vi "SMR_LabVIEW_V9.vi"() -> ()   [LabVIEW 2025]
uses:
  <vilib>/DAQmx/write.llb/DAQmx Write (Analog DBL 1Chan 1Samp).vi
  <vilib>/DAQmx/read.llb/DAQmx Read (Analog 1D DBL NChan 1Samp).vi
  <vilib>/DAQmx/read.llb/DAQmx Read (Analog 2D DBL NChan NSamp).vi
  <vilib>/Analysis/baseanly.llb/Mean (DBL).vi
  <vilib>/DAQmx/create/channels.llb/DAQmx Create Channel (AI-Temperature-Thermocouple).vi
  <vilib>/DAQmx/create/channels.llb/DAQmx Create Channel (AI-Voltage-Basic).vi
  <vilib>/DAQmx/create/channels.llb/DAQmx Create Channel (AO-Voltage-Basic).vi
  <vilib>/DAQmx/miscellaneous.llb/DAQmx Fill In Error Info.vi
  <vilib>/DAQmx/configure/timing.llb/DAQmx Timing (Sample Clock).vi
  <vilib>/addons/control/pid/pid.llb/PID (DBL).vi
  <vilib>/measure/maspectr.llb/FFT Power Spectrum and PSD for 1 Chan.vi
  <vilib>/measure/matone.llb/Extract Single Tone Information 1 Chan.vi
  <vilib>/addons/control/pid/NI_PID_pid.lvlib
  <vilib>/Analysis/NI_AALBase.lvlib
  <vilib>/ptbypt/NI_PtbyPt.lvlib
  <vilib>/measure/NI_MAPro.lvlib
panel:
  out "Room Temp (deg C)":dbl
  out "HW Valve Command (V)":dbl
  in  "HX Flow Setpoint (GPM)":dbl
  in  "Manual HW Valve Voltage (V)":dbl
  in  "HW Valve: Manual / PID":bool
  in  "PID gains for HW Valve":T1={"proportional gain (Kc)"=1.0, "integral time (Ti, min)"=0.01, "derivative time (Td, min)"=0.0} {"derivative time (Td, min)" format="%.3f"; "integral time (Ti, min)" format="%.3f"; "proportional gain (Kc)" format="%.3f"}
  out "Rod Power (W)":dbl
  out "Current Through Rod (A)":dbl
  out "Time in Steady State (s)":dbl
  in  "Steady-State Dwell (s)":dbl
  out "Main Loop Flow (GPM)":dbl
  out "FM Amplitude":dbl
  out "FM Frequency":dbl
  out "Spectrum":cluster{"f0":dbl, "df":dbl, "magnitude":dbl[]}(graph)
  out "Raw Signal":waveform(dbl)(graph)
  out "Smoothed HX Flow (GPM)":dbl
  out "Flow History":dbl(graph)
  out "HX Flow (GPM)":dbl
  out "Voltage Across Rod (V)":dbl format="%0.2f"
  out "Current Run Folder":path
  in  "Log Root Folder":path=path "C:/Users/LocalUser/Documents/GitHub/thermal-loop/resources/v0.1.1/data/001"
  out "Raw NI9201 \nVoltage Display":T2
  in  "Loop Period (ms)":dbl=1000.0
  in  "Stop":bool
  out "Auto Steady State Threshold (deg C/min)":dbl
  out "Max dT/dt (deg C/min)":dbl
  out "Temp Change Rate (deg C/min)":dbl
  out "5-Min Baseline Complete":bool
  out "Rate Window Ready":bool
  out "Steady State":bool
  in  "Voltage Limit (V)":dbl=10.0
  in  "Temperature Limit (C)":dbl=50.0
  in  "Pressure Limit (psi)":dbl=15.0
  out "Max Voltage":bool
  out "Max Temperature":bool
  out "Max Pressure":bool
  out "Heat Exchanger Pressure History":dbl(graph)
  out "Main Loop Pressure History":T3(graph)
  out "Overall Avg Pressure (psi)":dbl
  out "Heat Exchanger Pressure P6 (psi)":dbl
  out "Main Loop Avg Pressure (psi)":dbl
  out "Pressure Display":T4
  out "Overall Pressure History":T5(graph)
  out "Max Loop Pressure (psi)":dbl
  out "Heat Exchanger Temperature History":cluster{"Waveform":dbl, "Waveform":dbl}(graph)
  out "Main Loop Temeperature History":T6(graph)
  out "Heat Exchanger Avg Temp (deg C)":dbl
  out "Temperature Display":T7
  out "Overall Temperature History":T8(graph)
  out "Overall Avg Temp (deg C)":dbl
  out "Max Loop Temp (deg C)":dbl
  out "Final P-Valve Voltage (V)":dbl
  out "PID Trim Voltage (V)":dbl
  in  "PID Temp Setpoint (deg C)":dbl
  in  "Auto PID Enable":bool
  in  "Manual P-Valve Voltage (V)":dbl min=0.0 max=10.0
  out "Main Loop Avg Temp (deg C)":dbl
  # "HoneyWell Valve Control"
  # "Heat Exchanger Flow"
  # "Control/Troubleshoot"
  # "Steady State"
  # "Emergency Indicators"
  # "Pressure"
  # "Temperature"
  # "Proportional Valve Control"
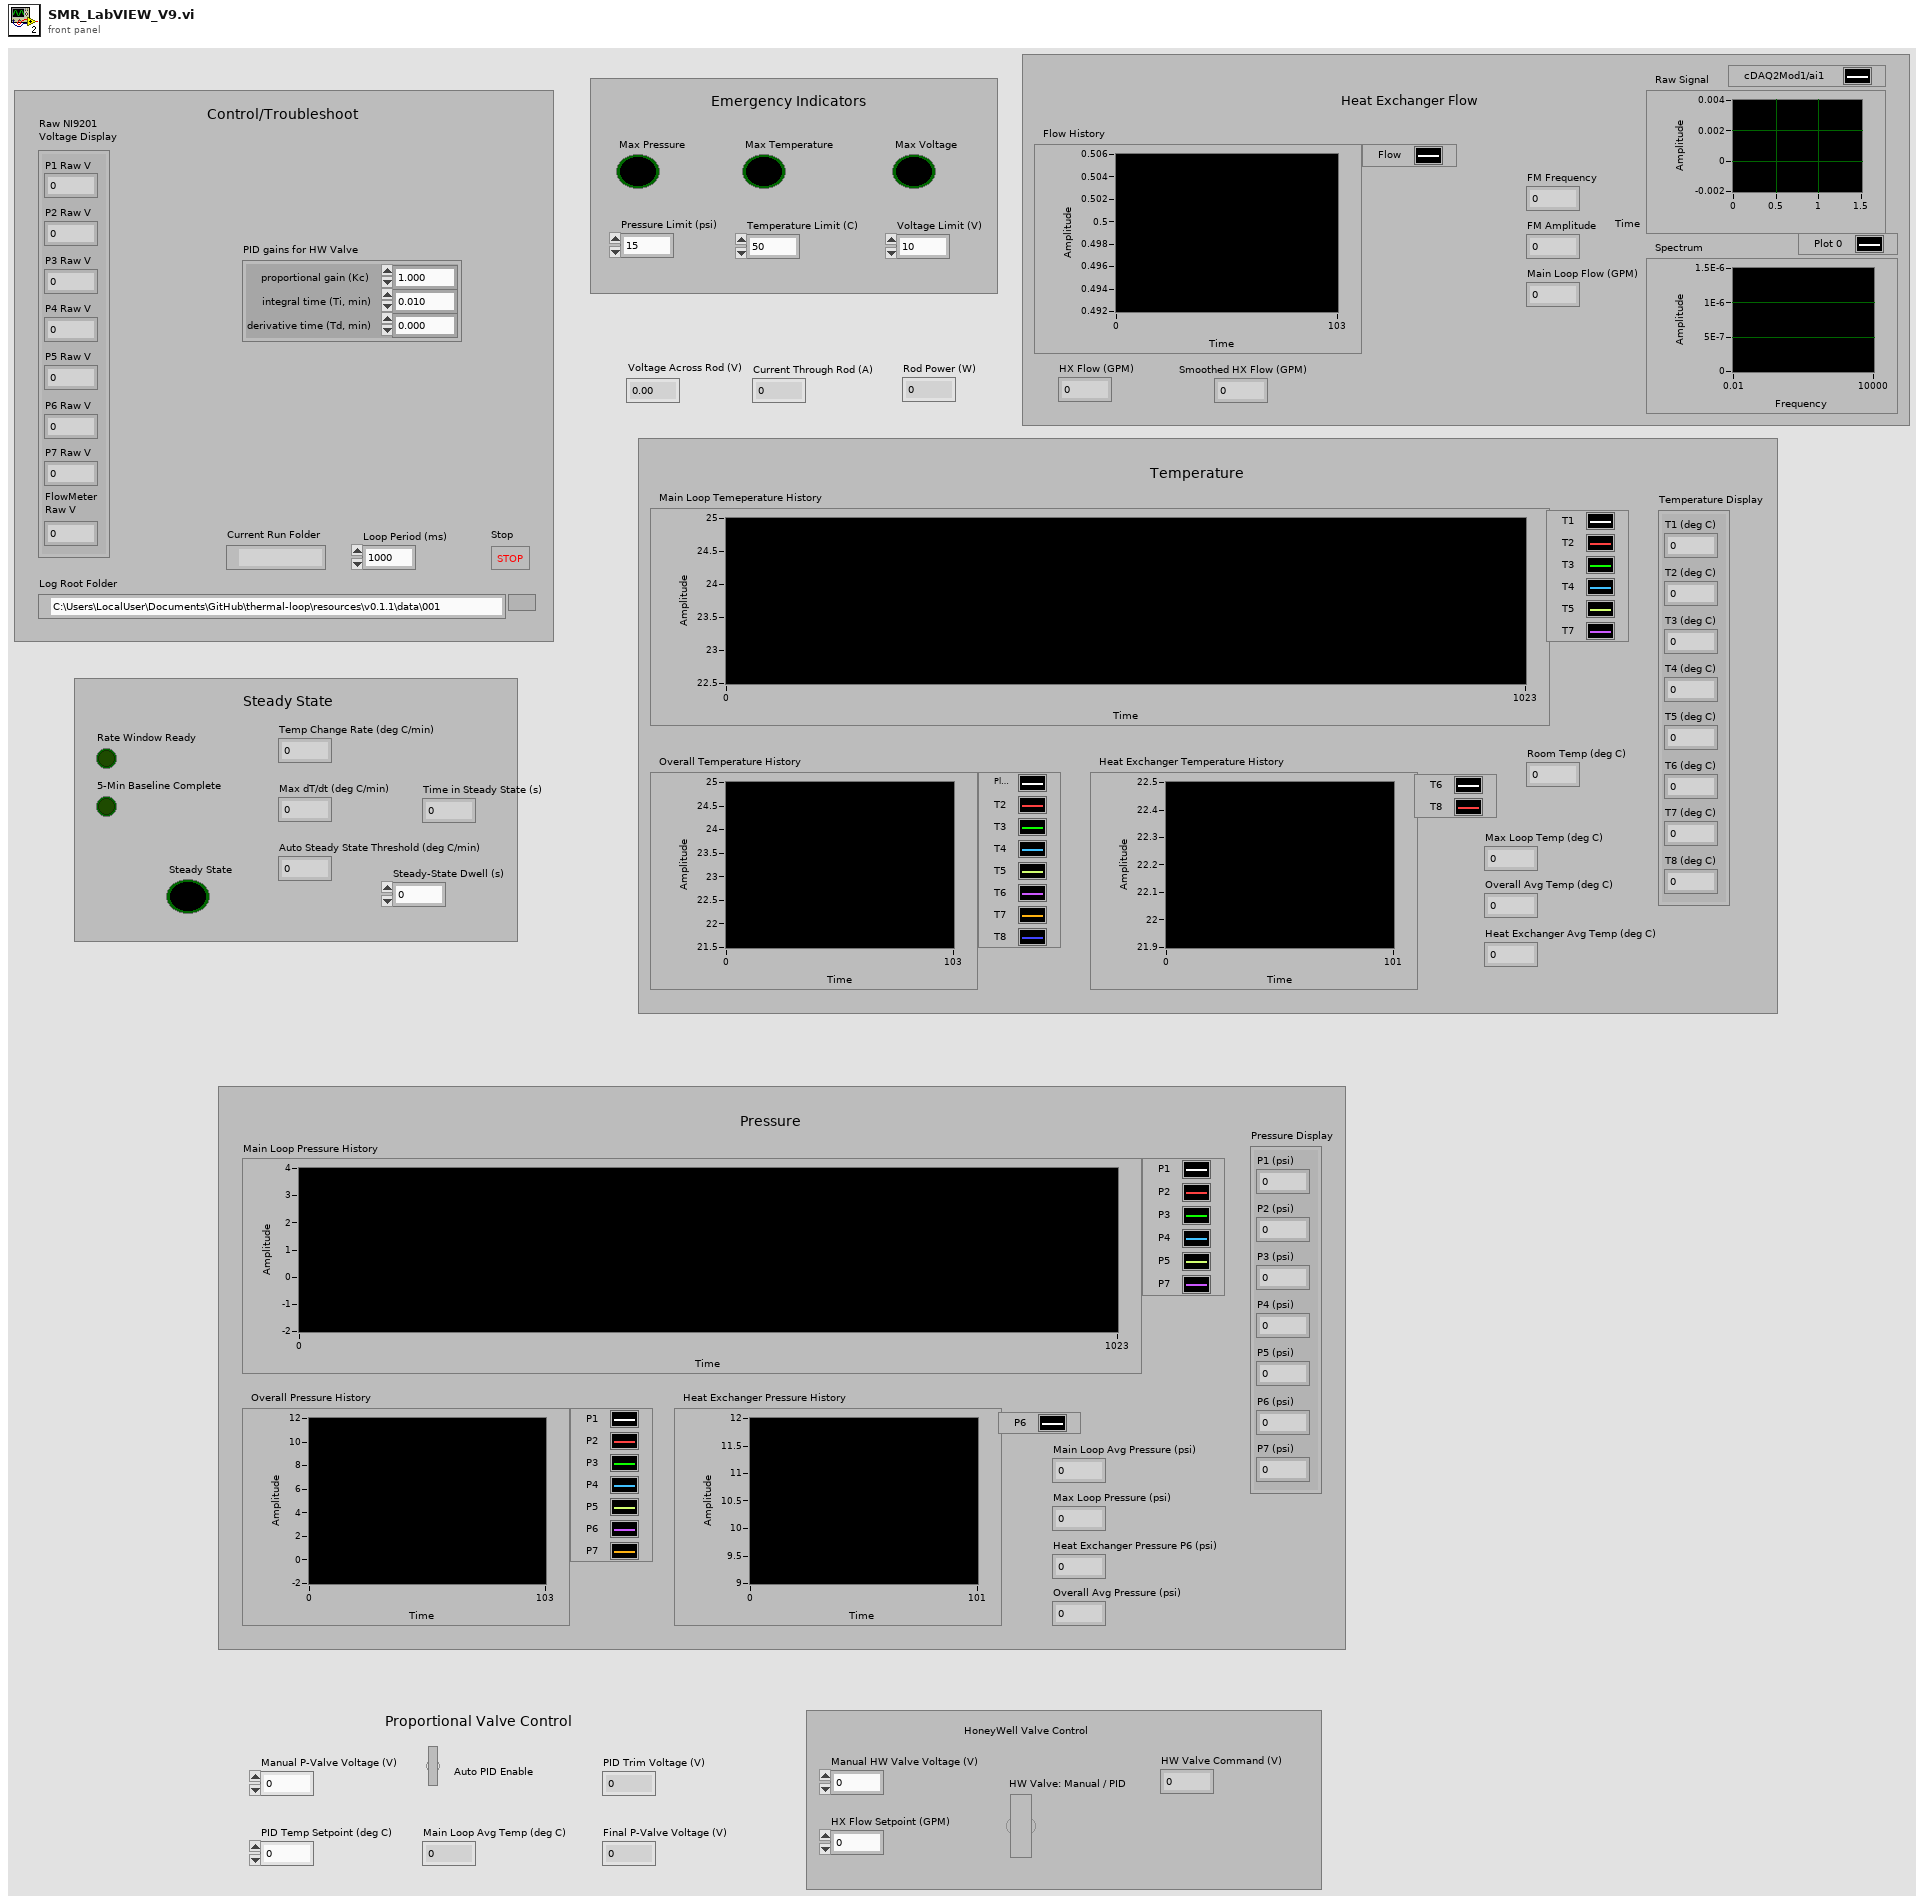
[diagram p1: front panel]
types:
  T1 = cluster{"proportional gain (Kc)":dbl, "integral time (Ti, min)":dbl, "derivative time (Td, min)":dbl}
  T2 = cluster{"P1 Raw V":dbl, "P2 Raw V":dbl, "P3 Raw V":dbl, "P4 Raw V":dbl, "P5 Raw V":dbl, "P6 Raw V":dbl, "P7 Raw V":dbl, "FlowMeter\nRaw V":dbl}
  T3 = cluster{"P1":dbl, "P2":dbl, "P3":dbl, "P4":dbl, "P5":dbl, "P7":dbl}
  T4 = cluster{"P1 (psi)":dbl, "P2 (psi)":dbl, "P3 (psi)":dbl, "P4 (psi)":dbl, "P5 (psi)":dbl, "P6 (psi)":dbl, "P7 (psi)":dbl}
  T5 = cluster{"P1":dbl, "P2":dbl, "P3":dbl, "P4":dbl, "P5":dbl, "P6":dbl, "P7":dbl}
  T6 = cluster{"Waveform":dbl, "Waveform":dbl, "Waveform":dbl, "Waveform":dbl, "Waveform":dbl, "Waveform":dbl}
  T7 = cluster{"T1 (deg C)":dbl, "T2 (deg C)":dbl, "T3 (deg C)":dbl, "T4 (deg C)":dbl, "T5 (deg C)":dbl, "T6 (deg C)":dbl, "T7 (deg C)":dbl, "T8 (deg C)":dbl}
  T8 = cluster{"Waveform":dbl, "Waveform":dbl, "Waveform":dbl, "Waveform":dbl, "Waveform":dbl, "Waveform":dbl, "Waveform":dbl, "Waveform":dbl}
  T9 = enum16{"open", "replace", "create", "open or create", "replace or create", "replace or create with confirmation"}
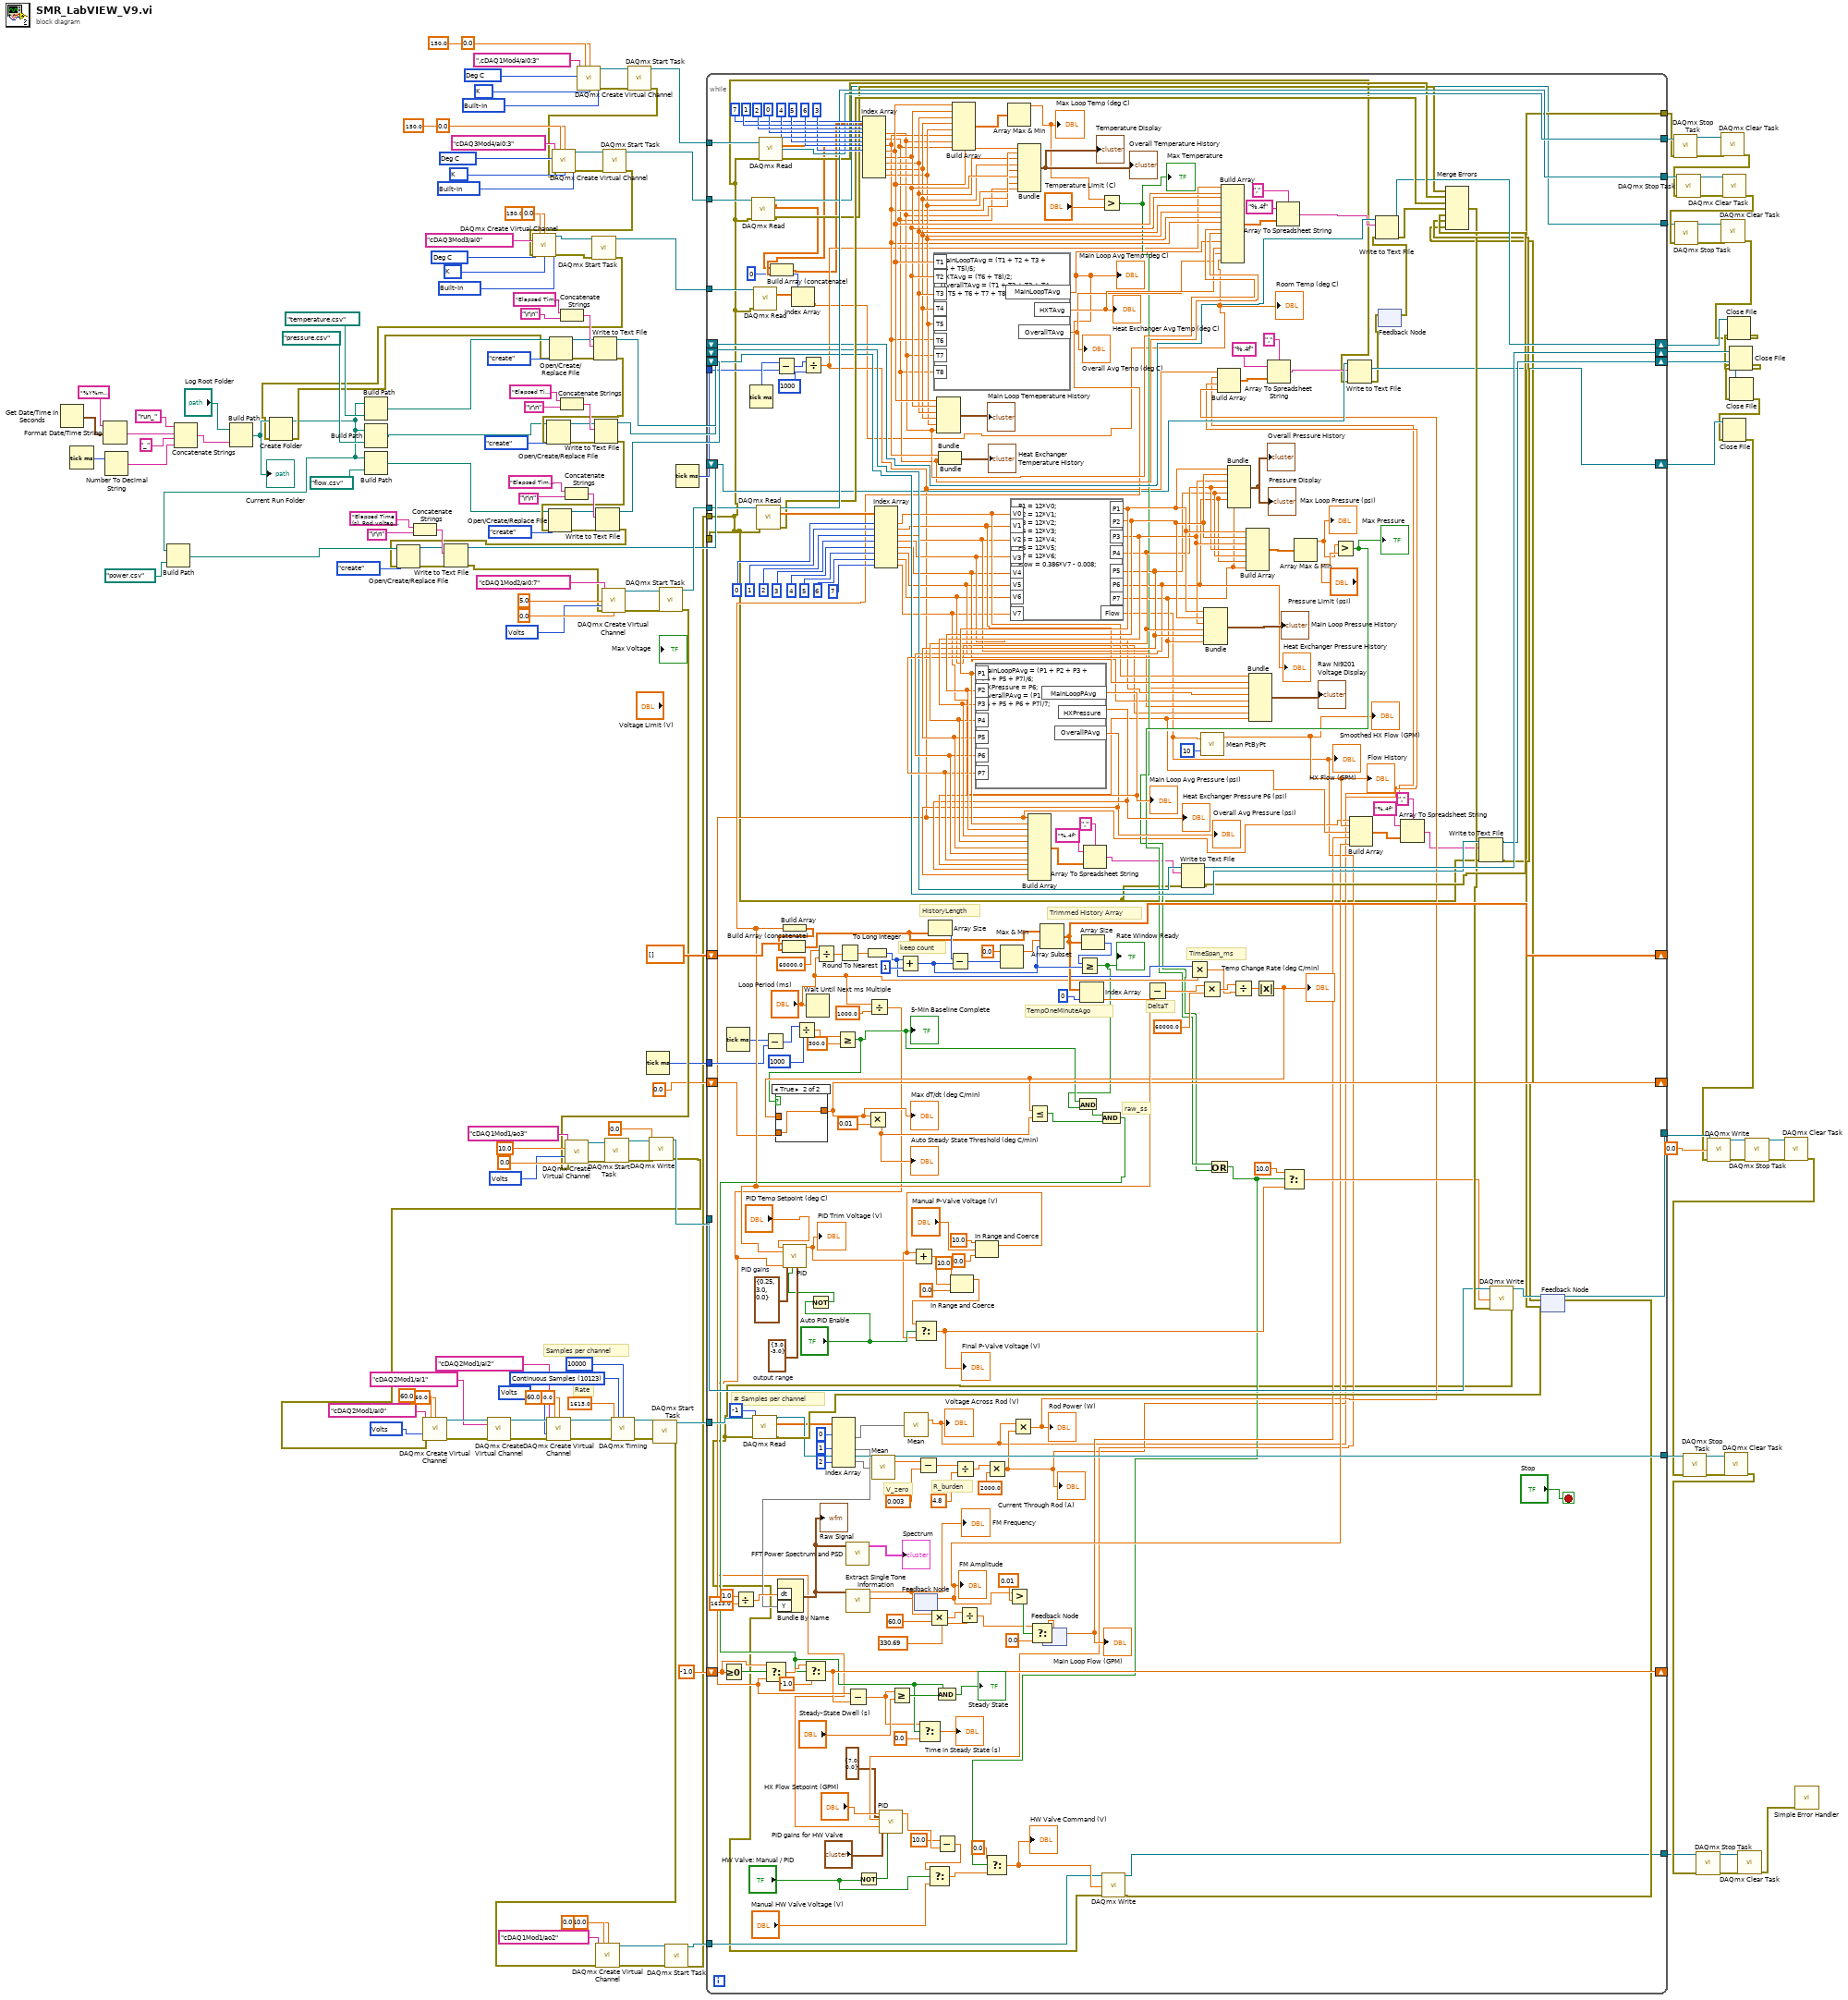
[diagram p0: block diagram]
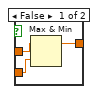
[diagram p2: hidden frame]
diagram:
  w1 = 10200 items=["Built-In"=10200, "Constant Value"=10116, "Channel"=10113] ("cjc source")
  w2 = 10073 items=["J"=10072, "K"=10073, "N"=10077, "R"=10082, "S"=10085, "T"=10086, "B"=10047, "E"=10055] ("thermocouple type")
  w8 = 10143 items=["Deg C"=10143, "Deg F"=10144, "Kelvins"=10325, "Deg R"=10145, "From Custom Scale"=10065] ("units")
  w28 = 10348 items=["Volts"=10348, "From Custom Scale"=10065] ("units")
  w44 = 10200 items=["Built-In"=10200, "Constant Value"=10116, "Channel"=10113] ("cjc source")
  w45 = 10073 items=["J"=10072, "K"=10073, "N"=10077, "R"=10082, "S"=10085, "T"=10086, "B"=10047, "E"=10055] ("thermocouple type")
  w46 = 10143 items=["Deg C"=10143, "Deg F"=10144, "Kelvins"=10325, "Deg R"=10145, "From Custom Scale"=10065] ("units")
  w76 = 10123 items=["Finite Samples"=10178, "Continuous Samples"=10123, "Hardware Timed Single Point"=12522] ("sample mode")
  w78 = 10348 items=["Volts"=10348, "From Custom Scale"=10065] ("units")
  w97 = 10348 items=["Volts"=10348, "From Custom Scale"=10065] ("units")
  w159 = 10200 items=["Built-In"=10200, "Constant Value"=10116, "Channel"=10113] ("cjc source")
  w160 = 10073 items=["J"=10072, "K"=10073, "N"=10077, "R"=10082, "S"=10085, "T"=10086, "B"=10047, "E"=10055] ("thermocouple type")
  w161 = 10143 items=["Deg C"=10143, "Deg F"=10144, "Kelvins"=10325, "Deg R"=10145, "From Custom Scale"=10065] ("units")
  w168 = 10348 items=["Volts"=10348, "From Custom Scale"=10065] ("units")
  # "Samples per channel"
  # "Rate"
  n1 = Get Date/Time In Seconds() -> (seconds since 1Jan1904=w118:timestamp)
  n2 = Tick Count (ms)() -> (millisecond timer value=w116:u32)
  n3 = Format Date/Time String(time format string (%c)="%Y%m%d_%H%M%S", seconds (now)=w118) -> (date/time string=w113:string)  [unwired: 1 in]
  n4 = Number To Decimal String(number=w116) -> (decimal integer string=w114:string)  [unwired: 1 in]
  n5 = Concatenate Strings("run_" ("string"), w113, "_" ("string"), w114) -> (w110:string)
  n6 = Build Path(base path="Log Root Folder", name or relative path=w110) -> (appended path=w109:path)
  "Current Run Folder" <- w109
  n7 = Concatenate Strings("Elapsed Time (s), Rod voltage (V), Rod Current (A), Rod Power (W)", "\r\n") -> (w63:string)
  n8 = Concatenate Strings("Elapsed Time (s),T1 (deg C),T2 (deg C),T3 (deg C),T4 (deg C),T5 (deg C),T6 (deg C),T7 (deg C),T8 (deg C),Main Loop Avg Temp (deg C),HX Avg Temp (deg C),Overall Avg Temp (deg C), Room Temp (deg C)", "\r\n") -> (w142:string)
  n9 = Concatenate Strings("Elapsed Time (s),P1 (psi),P2 (psi),P3 (psi),P4 (psi),P5 (psi),P6 (psi),P7 (psi),Main Loop Avg Pressure (psi),HX Pressure (psi),Overall Avg Pressure (psi)", "\r\n") -> (w140:string)
  n10 = Concatenate Strings("Elapsed Time (s),Heat Exchanger Flow (GPM),Flow Raw Voltage (V), Main Loop Flow (GPM), Flow Signal Amplitude (V)", "\r\n") -> (w136:string)
  n11 = call-poly <vilib>:"DAQmx Create Virtual Channel.vi"("maximum value"=150.0, "minimum value"=0.0, "physical channels"=tag ",cDAQ1Mod4/ai0:3", "cjc source"=w159, "units"=w161, "thermocouple type"=w160) -> ("task out"=w158:refnum<k21>, "error out"=w157:errorcluster)  [unwired: 8 in]
  n12 = call <vilib>:"DAQmx Start Task.vi"("task/channels in"=w158, "error in"=w157) -> ("task out"=w156:refnum<k21>, "error out"=w40:errorcluster)  [unwired: 12 in]
  n13 = call-poly <vilib>:"DAQmx Create Virtual Channel.vi"("maximum value"=150.0, "minimum value"=0.0, "physical channels"=tag "cDAQ3Mod4/ai0:3", "cjc source"=w44, "units"=w46, "error in"=w40, "thermocouple type"=w45) -> ("task out"=w43:refnum<k21>, "error out"=w42:errorcluster)  [unwired: 7 in]
  n14 = call <vilib>:"DAQmx Start Task.vi"("task/channels in"=w43, "error in"=w42) -> ("task out"=w39:refnum<k21>, "error out"=w5:errorcluster)  [unwired: 12 in]
  n15 = call-poly <vilib>:"DAQmx Create Virtual Channel.vi"("maximum value"=150.0, "minimum value"=0.0, "physical channels"=tag "cDAQ3Mod3/ai0", "cjc source"=w1, "units"=w8, "error in"=w5, "thermocouple type"=w2) -> ("task out"=w7:refnum<k21>, "error out"=w6:errorcluster)  [unwired: 7 in]
  n16 = call <vilib>:"DAQmx Start Task.vi"("task/channels in"=w7, "error in"=w6) -> ("task out"=w3:refnum<k21>, "error out"=w4:errorcluster)  [unwired: 12 in]
  n17 = Create Folder(path (use dialog)=w109, error in=w4) -> (created path=w57:path, error out=w102:errorcluster)  [unwired: 1 in, 1 out]
  n18 = Build Path(base path=w57, name or relative path=path "power.csv") -> (appended path=w58:path)
  n19 = Build Path(base path=w57, name or relative path=path "temperature.csv") -> (appended path=w108:path)
  n20 = Build Path(base path=w57, name or relative path=path "pressure.csv") -> (appended path=w107:path)
  n21 = Build Path(base path=w57, name or relative path=path "flow.csv") -> (appended path=w106:path)
  n22 = Open/Create/Replace File(file path (use dialog)=w108, error in=w102, operation (0:open)=T9."create") -> (refnum out=w141:refnum<file>, error out=w125:errorcluster)  [unwired: 3 in, 1 out]
  n23 = Write to Text File(file (use dialog)=w141, text=w142, error in=w125) -> (refnum out=w132:refnum<file>, error out=w124:errorcluster)  [unwired: 1 in, 1 out]
  n24 = Open/Create/Replace File(file path (use dialog)=w107, error in=w124, operation (0:open)=T9."create") -> (refnum out=w139:refnum<file>, error out=w123:errorcluster)  [unwired: 3 in, 1 out]
  n25 = Write to Text File(file (use dialog)=w139, text=w140, error in=w123) -> (refnum out=w131:refnum<file>, error out=w122:errorcluster)  [unwired: 1 in, 1 out]
  n26 = Open/Create/Replace File(file path (use dialog)=w106, error in=w122, operation (0:open)=T9."create") -> (refnum out=w135:refnum<file>, error out=w121:errorcluster)  [unwired: 3 in, 1 out]
  n27 = Write to Text File(file (use dialog)=w135, text=w136, error in=w121) -> (refnum out=w130:refnum<file>, error out=w55:errorcluster)  [unwired: 1 in, 1 out]
  n28 = Open/Create/Replace File(file path (use dialog)=w58, error in=w55, operation (0:open)=T9."create") -> (refnum out=w62:refnum<file>, error out=w59:errorcluster)  [unwired: 3 in, 1 out]
  n29 = Write to Text File(file (use dialog)=w62, text=w63, error in=w59) -> (refnum out=w53:refnum<file>, error out=w54:errorcluster)  [unwired: 1 in, 1 out]
  n30 = call-poly <vilib>:"DAQmx Create Virtual Channel.vi"("maximum value"=5.0, "minimum value"=0.0, "physical channels"=tag "cDAQ1Mod2/ai0:7", "units"=w168, "error in"=w54) -> ("task out"=w167:refnum<k21>, "error out"=w166:errorcluster)  [unwired: 9 in]
  n31 = Tick Count (ms)() -> (millisecond timer value=w83:u32)
  n32 = call <vilib>:"DAQmx Start Task.vi"("task/channels in"=w167, "error in"=w166) -> ("task out"=w165:refnum<k21>, "error out"=w90:errorcluster)  [unwired: 12 in]
  n33 = call-poly <vilib>:"DAQmx Create Virtual Channel.vi"("maximum value"=10.0, "minimum value"=0.0, "physical channels"=tag "cDAQ1Mod1/ao3", "units"=w97, "error in"=w90) -> ("task out"=w96:refnum<k21>, "error out"=w95:errorcluster)  [unwired: 9 in]
  n34 = call <vilib>:"DAQmx Start Task.vi"("task/channels in"=w96, "error in"=w95) -> ("task out"=w94:refnum<k21>, "error out"=w93:errorcluster)  [unwired: 12 in]
  n35 = call-poly <vilib>:"DAQmx Write.vi"("task/channels in"=w94, "data"=0.0, "error in"=w93) -> ("task out"=w91:refnum<k21>, "error out"=w70:errorcluster)  [unwired: 10 in, 1 out]
  n36 = call-poly <vilib>:"DAQmx Create Virtual Channel.vi"("maximum value"=60.0, "minimum value"=-60.0, "physical channels"=tag "cDAQ2Mod1/ai0", "units"=w78, "error in"=w70) -> ("task out"=w67:refnum<k21>, "error out"=w66:errorcluster)  [unwired: 9 in]
  n37 = call-poly <vilib>:"DAQmx Create Virtual Channel.vi"("task in"=w67, "physical channels"=tag "cDAQ2Mod1/ai1", "error in"=w66) -> ("task out"=w32:refnum<k21>, "error out"=w30:errorcluster)  [unwired: 11 in]
  n38 = call-poly <vilib>:"DAQmx Create Virtual Channel.vi"("task in"=w32, "maximum value"=60.0, "minimum value"=-60.0, "physical channels"=tag "cDAQ2Mod1/ai2", "units"=w28, "error in"=w30) -> ("task out"=w31:refnum<k21>, "error out"=w29:errorcluster)  [unwired: 8 in]
  n39 = call-poly <vilib>:"DAQmx Timing.vi"("task/channels in"=w31, "sample mode"=w76, "samples per channel"=10000, "rate"=1613.0, "error in"=w29) -> ("task out"=w74:refnum<k21>, "error out"=w73:errorcluster)  [unwired: 9 in]
  n40 = call <vilib>:"DAQmx Start Task.vi"("task/channels in"=w74, "error in"=w73) -> ("task out"=w69:refnum<k21>, "error out"=w19:errorcluster)  [unwired: 12 in]
  n41 = call-poly <vilib>:"DAQmx Create Virtual Channel.vi"("maximum value"=10.0, "minimum value"=0.0, "physical channels"=tag "cDAQ1Mod1/ao2", "error in"=w19) -> ("task out"=w22:refnum<k21>, "error out"=w21:errorcluster)  [unwired: 10 in]
  n42 = call <vilib>:"DAQmx Start Task.vi"("task/channels in"=w22, "error in"=w21) -> ("task out"=w20:refnum<k21>, "error out"=w18:errorcluster)  [unwired: 12 in]
  n43 = Tick Count (ms)() -> (millisecond timer value=w129:u32)
  n44 = while {
    tunnel: w165 -> [w411]
    tunnel: w156 -> [w394]
    tunnel: [w385] -> w155
    tunnel: [w175] -> _
    tunnel: [w384] -> w154
    tunnel: [w272] -> w153
    shift-right: [w363] -> w128
    shift-left: w132 -> [w364]
    shift-right: [w348] -> w127
    shift-left: w131 -> [w349]
    shift-right: [w343] -> w126
    shift-left: w130 -> [w344]
    tunnel: w129 -> [w380]
    shift-right: [w322] -> _
    shift-left: dbl[] [] -> [w335]
    tunnel: w91 -> [w304]
    tunnel: w18 -> [w175]
    tunnel: [w310] -> w88
    tunnel: w83 -> [w293]
    shift-right: [w286] -> _
    shift-left: 0.0 -> [w288]
    tunnel: w69 -> [w271]
    tunnel: [w270] -> w68
    shift-right: [w233] -> w52
    shift-left: w53 -> [w234]
    shift-right: [w225] -> _
    shift-left: -1.0 -> [w229]
    tunnel: w39 -> [w217]
    tunnel: [w215] -> w35
    tunnel: w20 -> [w194]
    tunnel: [w190] -> w13
    tunnel: w3 -> [w176]
    stop <- "Stop" stop-if-true
    w308 = cluster{"output high":dbl, "output low":dbl} {"output high"=3.0, "output low"=-3.0}  # output range
    w309 = T1 {"proportional gain (Kc)"=0.25, "integral time (Ti, min)"=3.0, "derivative time (Td, min)"=0.0}  # PID gains
    # "R_burden"
    # "V_zero"
    # "raw_ss"
    # "# Samples per channel"
    # "TimeSpan_ms"
    # "DeltaT"
    # "TempOneMinuteAgo"
    # "Trimmed History Array"
    # "HistoryLength"
    # "keep count"
    n45 = Greater Or Equal To 0?(x=w229) -> (x >= 0?=w230:bool)
    n46 = Tick Count (ms)() -> (millisecond timer value=w294:u32)
    n47 = Divide(x=1.0, y=1613.0) -> (x/y=w244:dbl)
    n48 = Tick Count (ms)() -> (millisecond timer value=w381:u32)
    n49 = call-poly <vilib>:"DAQmx Read.vi"("task/channels in"=w217, "error in"=w175) -> ("task out"=w215:refnum<k21>, "data"=w212:dbl[], "error out"=w216:errorcluster)  [unwired: 11 in]
    n50 = call-poly <vilib>:"DAQmx Read.vi"("task/channels in"=w176, "error in"=w175) -> ("data"=w173:dbl[])  [unwired: 11 in, 2 out]
    n51 = call-poly <vilib>:"DAQmx Read.vi"("task/channels in"=w411, "error in"=w175) -> ("task out"=w384:refnum<k21>, "data"=w402:dbl[], "error out"=w382:errorcluster)  [unwired: 11 in]
    n52 = call-poly <vilib>:"DAQmx Read.vi"("task/channels in"=w394, "error in"=w175) -> ("task out"=w385:refnum<k21>, "data"=w213:dbl[], "error out"=w383:errorcluster)  [unwired: 11 in]
    n53 = Subtract(x=w294, y=w293) -> (x-y=w292:u32)
    n54 = Build Array (concatenate)(w212, w213) -> (w214:dbl[])
    n55 = Subtract(x=w381, y=w380) -> (x-y=w379:u32)
    n56 = Index Array(array=w173, index=0) -> (element=w172:dbl)
    "Room Temp (deg C)" <- w172
    n57 = Divide(x=w292, y=u32 1000) -> (x/y=w290:dbl)
    n58 = Divide(x=w379, y=u32 1000) -> (x/y=w226:dbl)
    n59 = Select(t=w229, s=w230, f=w226) -> (s? t:f=w228:dbl)
    n60 = Wait Until Next ms Multiple(millisecond multiple="Loop Period (ms)") -> ()  [unwired: 1 out]
    n61 = Not(x="Auto PID Enable") -> (.not. x?=w305:bool)
    n62 = Divide(x=60000.0, y="Loop Period (ms)") -> (x/y=w332:dbl)
    n63 = Greater Or Equal?(x=w290, y=300.0) -> (x >= y?=w283:bool)
    "5-Min Baseline Complete" <- w283
    n64 = Round To Nearest(number=w332) -> (nearest integer value=w331:dbl)
    n65 = Not(x="HW Valve: Manual / PID") -> (.not. x?=w204:bool)
    n66 = Index Array(array=w214, index #1=7 ("index"), index #2=1 ("index"), index #3=2 ("index"), index #4=0 ("index"), index #5=4 ("index"), index #6=5 ("index"), index #7=6 ("index"), index #8=3 ("index")) -> (element #1=w371:dbl, element #2=w370:dbl, element #3=w372:dbl, element #4=w377:dbl, element #5=w376:dbl, element #6=w375:dbl, element #7=w374:dbl, element #8=w373:dbl)
    n67 = To Long Integer(number=w331) -> (32bit integer=w319:i32)
    n68 = Divide(x="Loop Period (ms)", y=1000.0) -> (x/y=w189:dbl)
    n69 = Index Array(array=w402, index #1=0 ("index"), index #2=1 ("index"), index #3=2 ("index"), index #4=3 ("index"), index #5=4 ("index"), index #6=5 ("index"), index #7=6 ("index"), index #8=7 ("index")) -> (element #1=w269:dbl, element #2=w268:dbl, element #3=w267:dbl, element #4=w266:dbl, element #5=w265:dbl, element #6=w264:dbl, element #7=w263:dbl, element #8=w262:dbl)
    n70 = Add(x=w319, y=1) -> (x+y=w324:i32)
    n71 = feedback #1() -> (w240:dbl)  [unwired: 1 in]
    "FM Amplitude" <- w240
    n72 = formula code="MainLoopTAvg = (T1 + T2 + T3 + T4 + T5)/5;\nHXTAvg = (T6 + T8)/2;\nOverallTAvg = (T1 + T2 + T3 + T4 + T5 + T6 + T7 + T8)/8;"("T1"=w377, "T2"=w376, "T3"=w375, "T4"=w374, "T5"=w373, "T6"=w372, "T7"=w371, "T8"=w370) -> ("MainLoopTAvg"=w296:dbl, "HXTAvg"=w369:dbl, "OverallTAvg"=w368:dbl)
    "Overall Avg Temp (deg C)" <- w368
    "Main Loop Avg Temp (deg C)" <- w296
    "Heat Exchanger Avg Temp (deg C)" <- w369
    n73 = Build Array(w296) -> (w334:dbl[])
    n74 = Build Array (concatenate)(w335, w334) -> (w326:dbl[])
    n75 = call-poly <vilib>:"PID.vi"("reinitialize? (F)"=w305, "output range"=w308, "dt (s)"=w189, "PID gains"=w309, "process variable"=w296, "setpoint"="PID Temp Setpoint (deg C)") -> ("output"=w303:dbl)  [unwired: 4 in, 1 out]
    "PID Trim Voltage (V)" <- w303
    n76 = Array Size(array=w326) -> (size(s)=w329:i32)
    n77 = Bundle("Waveform"=w377, "Waveform"=w376, "Waveform"=w375, "Waveform"=w374, "Waveform"=w373, "Waveform"=w371) -> (→"Main Loop Temeperature History":T6)  [unwired: 1 in]
    n78 = Bundle("Waveform"=w372, "Waveform"=w370) -> (→"Heat Exchanger Temperature History":cluster{"Waveform":dbl, "Waveform":dbl})  [unwired: 1 in]
    n79 = Subtract(x=w329, y=w324) -> (x-y=w327:i32)
    n80 = Build Array(w377, w376, w375, w374, w373, w372, w371, w370) -> (w412:dbl[])
    n81 = In Range and Coerce(upper limit=10.0, x="Manual P-Valve Voltage (V)", lower limit=0.0) -> (coerced(x)=w298:dbl)  [unwired: 1 out]
    n82 = Add(x=w298, y=w303) -> (x+y=w302:dbl)
    n83 = In Range and Coerce(upper limit=10.0, x=w302, lower limit=0.0) -> (coerced(x)=w297:dbl)  [unwired: 1 out]
    n84 = Select(t=w297, s="Auto PID Enable", f=w298) -> (s? t:f=w275:dbl)
    "Final P-Valve Voltage (V)" <- w275
    n85 = Max & Min(x=0.0, y=w327) -> (max(x,y)=w325:dbl)  [unwired: 1 out]
    n86 = Array Max & Min(array=w412) -> (max value=w337:dbl)  [unwired: 3 out]
    "Max Loop Temp (deg C)" <- w337
    n87 = Greater?(x=w240, y=0.01) -> (0:w248:bool)
    n88 = formula code="P1 = 12*V0;\nP2 = 12*V1;\nP3 = 12*V2;\nP4 = 12*V3;\nP5 = 12*V4;\nP6 = 12*V5; \nP7 = 12*V6;\nFlow = 0.386*V7 - 0.008;"("V0"=w269, "V1"=w268, "V2"=w267, "V3"=w266, "V4"=w265, "V5"=w264, "V6"=w263, "V7"=w262) -> ("P1"=w362:dbl, "P2"=w361:dbl, "P3"=w360:dbl, "P4"=w359:dbl, "P5"=w358:dbl, "P6"=w357:dbl, "P7"=w356:dbl, "Flow"=w207:dbl)
    "HX Flow (GPM)" <- w207
    "Heat Exchanger Pressure History" <- w357
    n89 = call-poly <vilib>:"PID.vi"("reinitialize? (F)"=w204, "output range"=cluster{"output high":dbl, "output low":dbl} {"output high"=7.0, "output low"=0.0}, "dt (s)"=w189, "PID gains"="PID gains for HW Valve", "process variable"=w207, "setpoint"="HX Flow Setpoint (GPM)") -> ("output"=w203:dbl)  [unwired: 4 in, 1 out]
    n90 = Subtract(x=10.0, y=w203) -> (x-y=w200:dbl)
    n91 = Select(t=w200, s="HW Valve: Manual / PID", f="Manual HW Valve Voltage (V)") -> (s? t:f=w197:dbl)
    n92 = formula code="MainLoopPAvg = (P1 + P2 + P3 + P4 + P5 + P7)/6;\nHXPressure = P6;\nOverallPAvg = (P1 + P2 + P3 + P4 + P5 + P6 + P7)/7;"("P1"=w362, "P2"=w361, "P3"=w360, "P4"=w359, "P5"=w358, "P6"=w357, "P7"=w356) -> ("MainLoopPAvg"=w355:dbl, "HXPressure"=w354:dbl, "OverallPAvg"=w353:dbl)
    "Overall Avg Pressure (psi)" <- w353
    "Heat Exchanger Pressure P6 (psi)" <- w354
    "Main Loop Avg Pressure (psi)" <- w355
    n93 = Bundle("Waveform"=w377, "Waveform"=w376, "Waveform"=w375, "Waveform"=w374, "Waveform"=w373, "Waveform"=w372, "Waveform"=w371, "Waveform"=w370) -> (→"Overall Temperature History" →"Temperature Display":T8)  [unwired: 1 in]
    n94 = Build Array(w226, w362, w361, w360, w359, w358, w357, w356, w355, w354, w353) -> (w352:dbl[])
    n95 = Array Subset(array=w326, index=w325, length=w324) -> (w322:dbl[])
    n96 = feedback #2() -> (w238:dbl)  [unwired: 1 in]
    "Main Loop Flow (GPM)" <- w238
    n97 = Index Array(array=w322, index=0) -> (element=w320:dbl)
    n98 = Array Size(array=w322) -> (size(s)=w323:i32)
    n99 = Greater Or Equal?(x=w323, y=w324) -> (x >= y?=w282:bool)
    "Rate Window Ready" <- w282
    n100 = And(x=w283, y=w282) -> (x .and. y?=w281:bool)
    n101 = Array To Spreadsheet String(delimiter (Tab)=",", array=w352, 3:"%.4f" ("format string")) -> (spreadsheet string=w185:string)
    n102 = Greater?(x=w337, y="Temperature Limit (C)") -> (0:w278:bool)
    "Max Temperature" <- w278
    n103 = Subtract(x=w296, y=w320) -> (x-y=w318:dbl)
    n104 = Write to Text File(file (use dialog)=w349, text=w185, error in=w175) -> (refnum out=w348:refnum<file>, error out=w341:errorcluster)  [unwired: 1 in, 1 out]
    n105 = Multiply(x=w319, y="Loop Period (ms)") -> (x*y=w315:dbl)
    n106 = Multiply(x=w318, y=60000.0) -> (x*y=w316:dbl)
    n107 = call <vilib>:"Mean PtByPt.vi"("x"=w207, "sample length"=10) -> ("mean"=w260:dbl)  [unwired: 2 in, 1 out]
    "Flow History" <- w260
    "Smoothed HX Flow (GPM)" <- w260
    n108 = Bundle("P1"=w362, "P2"=w361, "P3"=w360, "P4"=w359, "P5"=w358, "P7"=w356) -> (→"Main Loop Pressure History":T3)  [unwired: 1 in]
    n109 = Build Array(w226, w377, w376, w375, w374, w373, w372, w371, w370, w296, w369, w368, w172) -> (w367:dbl[])
    n110 = Bundle("P1"=w362, "P2"=w361, "P3"=w360, "P4"=w359, "P5"=w358, "P6"=w357, "P7"=w356) -> (→"Overall Pressure History" →"Pressure Display":T5)  [unwired: 1 in]
    n111 = Divide(x=w316, y=w315) -> (x/y=w314:dbl)
    n112 = Build Array(w362, w361, w360, w359, w358, w357, w356) -> (w401:dbl[])
    n113 = Bundle("Waveform"=w269, "Waveform"=w268, "Waveform"=w267, "Waveform"=w266, "Waveform"=w265, "Waveform"=w264, "Waveform"=w263, "Waveform"=w262) -> (→"Raw NI9201 \nVoltage Display":T8)  [unwired: 1 in]
    n114 = Absolute Value(x=w314) -> (abs(x)=w285:dbl)
    "Temp Change Rate (deg C/min)" <- w285
    n115 = case shown="True" w283 {
      tunnel: w288 -> [w416 w417]
      tunnel: w285 -> [w415 _]
      tunnel: [w414 w417] -> w286
      frame False {
        n116 = Max & Min(x=w415, y=w416) -> (max(x,y)=w414:dbl)  [unwired: 1 out]
      }
      frame True {
      }
    }
    "Max dT/dt (deg C/min)" <- w286
    n117 = Multiply(x=w286, y=0.01) -> (x*y=w284:dbl)
    "Auto Steady State Threshold (deg C/min)" <- w284
    n118 = Less Or Equal?(x=w285, y=w284) -> (x <= y?=w280:bool)
    n119 = And(x=w281, y=w280) -> (x .and. y?=w221:bool)
    n120 = Select(t=w228, s=w221, f=-1.0) -> (s? t:f=w225:dbl)
    n121 = Subtract(x=w226, y=w225) -> (x-y=w220:dbl)
    n122 = Greater Or Equal?(x=w220, y="Steady-State Dwell (s)") -> (x >= y?=w223:bool)
    n123 = Select(t=w220, s=w221, f=0.0) -> (s? t:f=→"Time in Steady State (s)":dbl)
    n124 = And(x=w221, y=w223) -> (x .and. y?=→"Steady State":bool)
    n125 = Array To Spreadsheet String(delimiter (Tab)=",", array=w367, 3:"%.4f" ("format string")) -> (spreadsheet string=w186:string)
    n126 = Array Max & Min(array=w401) -> (max value=w338:dbl)  [unwired: 3 out]
    "Max Loop Pressure (psi)" <- w338
    n127 = Greater?(x=w338, y="Pressure Limit (psi)") -> (0:w279:bool)
    "Max Pressure" <- w279
    n128 = Or(x=w279, y=w278) -> (x .or. y?=w198:bool)
    n129 = Select(t=0.0, s=w198, f=w197) -> (s? t:f=w195:dbl)
    "HW Valve Command (V)" <- w195
    n130 = Select(t=10.0, s=w198, f=w275) -> (s? t:f=w274:dbl)
    n131 = Build Array(w226, w260, w262, w238, w240) -> (w347:dbl[])
    n132 = feedback #3() -> (w231:errorcluster)  [unwired: 1 in]
    n133 = Write to Text File(file (use dialog)=w364, text=w186, error in=w231) -> (refnum out=w363:refnum<file>, error out=w342:errorcluster)  [unwired: 1 in, 1 out]
    n134 = Array To Spreadsheet String(delimiter (Tab)=",", array=w347, 3:"%.4f" ("format string")) -> (spreadsheet string=w188:string)
    n135 = Write to Text File(file (use dialog)=w344, text=w188, error in=w175) -> (refnum out=w343:refnum<file>, error out=w340:errorcluster)  [unwired: 1 in, 1 out]
    n136 = feedback #4() -> (w191:errorcluster)  [unwired: 1 in]
    n137 = Merge Errors(w216, w383, w382, w342, w341, w340, w191) -> (w311:errorcluster)
    n138 = call-poly <vilib>:"DAQmx Write.vi"("task/channels in"=w304, "data"=w274, "error in"=w311) -> ("task out"=w310:refnum<k21>, "error out"=w193:errorcluster)  [unwired: 10 in, 1 out]
    n139 = call-poly <vilib>:"DAQmx Read.vi"("task/channels in"=w271, "number of samples per channel"=-1, "error in"=w193) -> ("task out"=w270:refnum<k21>, "data"=w259:dbl[][], "error out"=w272:errorcluster)  [unwired: 10 in]
    n140 = Index Array(array=w259, index (row) #1=0 ("index (row)"), index (row) #2=1 ("index (row)"), index (row) #3=2 ("index (row)")) -> (element #1=w258:dbl[], element #2=w243:dbl[], element #3=w210:dbl[])  [unwired: 3 in]
    n141 = Bundle By Name("dt"=w244, "Y"=w243) -> (w242:waveform(dbl))  [unwired: 1 in]
    "Raw Signal" <- w242
    n142 = call-poly <vilib>:"FFT Power Spectrum and PSD.vi"("time signal"=w242) -> ("Power Spectrum / PSD"=→"Spectrum":cluster{"f0":dbl, "df":dbl, "magnitude":dbl[]})  [unwired: 7 in, 3 out]
    n143 = call-poly <vilib>:"Extract Single Tone Information.vi"("time signal in"=w242) -> ("detected amplitude"=w241:dbl, "detected frequency"=w254:dbl)  [unwired: 5 in, 4 out]
    "FM Frequency" <- w254
    n144 = call-poly <vilib>:"Mean.vi"("X"=w210) -> ("mean"=w184:dbl)  [unwired: 1 out]
    n145 = call-poly <vilib>:"Mean.vi"("X"=w258) -> ("mean"=w177:dbl)  [unwired: 1 out]
    "Voltage Across Rod (V)" <- w177
    n146 = feedback-in #1(w241) -> ()
    n147 = Subtract(x=w184, y=0.003) -> (x-y=w182:dbl)
    n148 = Multiply(x=w254, y=60.0) -> (x*y=w252:dbl)
    n149 = Divide(x=w182, y=4.8) -> (x/y=w180:dbl)
    n150 = Divide(x=w252, y=330.69) -> (x/y=w247:dbl)
    n151 = Multiply(x=w180, y=2000.0) -> (x*y=w178:dbl)
    "Current Through Rod (A)" <- w178
    n152 = Multiply(x=w177, y=w178) -> (x*y=w209:dbl)
    "Rod Power (W)" <- w209
    n153 = Select(t=w247, s=w248, f=0.0) -> (s? t:f=w239:dbl)
    n154 = feedback-in #2(w239) -> ()
    n155 = call-poly <vilib>:"DAQmx Write.vi"("task/channels in"=w194, "data"=w195, "error in"=w193) -> ("task out"=w190:refnum<k21>, "error out"=w192:errorcluster)  [unwired: 10 in, 1 out]
    n156 = Build Array(w226, w177, w178, w209) -> (w235:dbl[])
    n157 = Array To Spreadsheet String(delimiter (Tab)=",", array=w235, 3:"%.4f" ("format string")) -> (spreadsheet string=w187:string)
    n158 = Write to Text File(file (use dialog)=w234, text=w187, error in=w175) -> (refnum out=w233:refnum<file>, error out=w232:errorcluster)  [unwired: 1 in, 1 out]
    n159 = feedback-in #3(w232) -> ()
    n160 = feedback-in #4(w192) -> ()
  }
  n161 = call <vilib>:"DAQmx Stop Task.vi"("task/channels in"=w155, "error in"=w153) -> ("task out"=w152:refnum<k21>, "error out"=w150:errorcluster)  [unwired: 12 in]
  n162 = call <vilib>:"DAQmx Clear Task.vi"("task in"=w152, "error in"=w150) -> ("error out"=w149:errorcluster)  [unwired: 13 in]
  n163 = call <vilib>:"DAQmx Stop Task.vi"("task/channels in"=w154, "error in"=w149) -> ("task out"=w151:refnum<k21>, "error out"=w148:errorcluster)  [unwired: 12 in]
  n164 = call <vilib>:"DAQmx Clear Task.vi"("task in"=w151, "error in"=w148) -> ("error out"=w38:errorcluster)  [unwired: 13 in]
  n165 = call <vilib>:"DAQmx Stop Task.vi"("task/channels in"=w35, "error in"=w38) -> ("task out"=w34:refnum<k21>, "error out"=w37:errorcluster)  [unwired: 12 in]
  n166 = call <vilib>:"DAQmx Clear Task.vi"("task in"=w34, "error in"=w37) -> ("error out"=w36:errorcluster)  [unwired: 13 in]
  n167 = Close File(refnum=w128, error in=w36) -> (error out=w120:errorcluster)  [unwired: 1 out]
  n168 = Close File(refnum=w127, error in=w120) -> (error out=w119:errorcluster)  [unwired: 1 out]
  n169 = Close File(refnum=w126, error in=w119) -> (error out=w51:errorcluster)  [unwired: 1 out]
  n170 = Close File(refnum=w52, error in=w51) -> (error out=w50:errorcluster)  [unwired: 1 out]
  n171 = call-poly <vilib>:"DAQmx Write.vi"("task/channels in"=w88, "data"=0.0, "error in"=w50) -> ("task out"=w87:refnum<k21>, "error out"=w85:errorcluster)  [unwired: 10 in, 1 out]
  n172 = call <vilib>:"DAQmx Stop Task.vi"("task/channels in"=w87, "error in"=w85) -> ("task out"=w86:refnum<k21>, "error out"=w84:errorcluster)  [unwired: 12 in]
  n173 = call <vilib>:"DAQmx Clear Task.vi"("task in"=w86, "error in"=w84) -> ("error out"=w17:errorcluster)  [unwired: 13 in]
  n174 = call <vilib>:"DAQmx Stop Task.vi"("task/channels in"=w68, "error in"=w17) -> ("task out"=w72:refnum<k21>, "error out"=w71:errorcluster)  [unwired: 12 in]
  n175 = call <vilib>:"DAQmx Clear Task.vi"("task in"=w72, "error in"=w71) -> ("error out"=w14:errorcluster)  [unwired: 13 in]
  n176 = call <vilib>:"DAQmx Stop Task.vi"("task/channels in"=w13, "error in"=w14) -> ("task out"=w16:refnum<k21>, "error out"=w15:errorcluster)  [unwired: 12 in]
  n177 = call <vilib>:"DAQmx Clear Task.vi"("task in"=w16, "error in"=w15) -> ("error out"=w12:errorcluster)  [unwired: 13 in]
  n178 = call <vilib>:"Simple Error Handler.vi"("error in (no error)"=w12) -> ()  [unwired: 4 in, 5 out]
